vi "Test - Add  Property (Array).vi"() -> ()   [LabVIEW 2020, in "JSON Schema Generator.lvlib"]
uses:
  JSON Schema Generator.lvlib
  <vilib>/addons/_JKI Toolkits/Caraya/classes/Test/Test.lvclass
  <vilib>/addons/_JKI Toolkits/Caraya/classes/Assert/Assert.lvclass
  <vilib>/JDP Science/JSONtext/JSONtext.lvlib
  <vilib>/addons/_JKI Toolkits/Caraya/classes/Assert/Assert Equal Value_Variant.vi
  <vilib>/addons/_JKI Toolkits/Caraya/classes/Assert/Assert Not Error.vi
panel:
  in  "Array 3":enum16{"Test 1", "Test 2", "Test3"}[](array[ring])
  in  "Array 2":string[](array[string])
  in  "Array":T1(array[cluster])
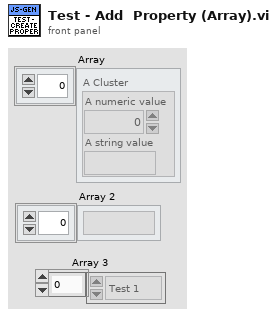
[diagram p1: front panel]
types:
  T1 = cluster{"A numeric value":i32, "A string value":string}[]
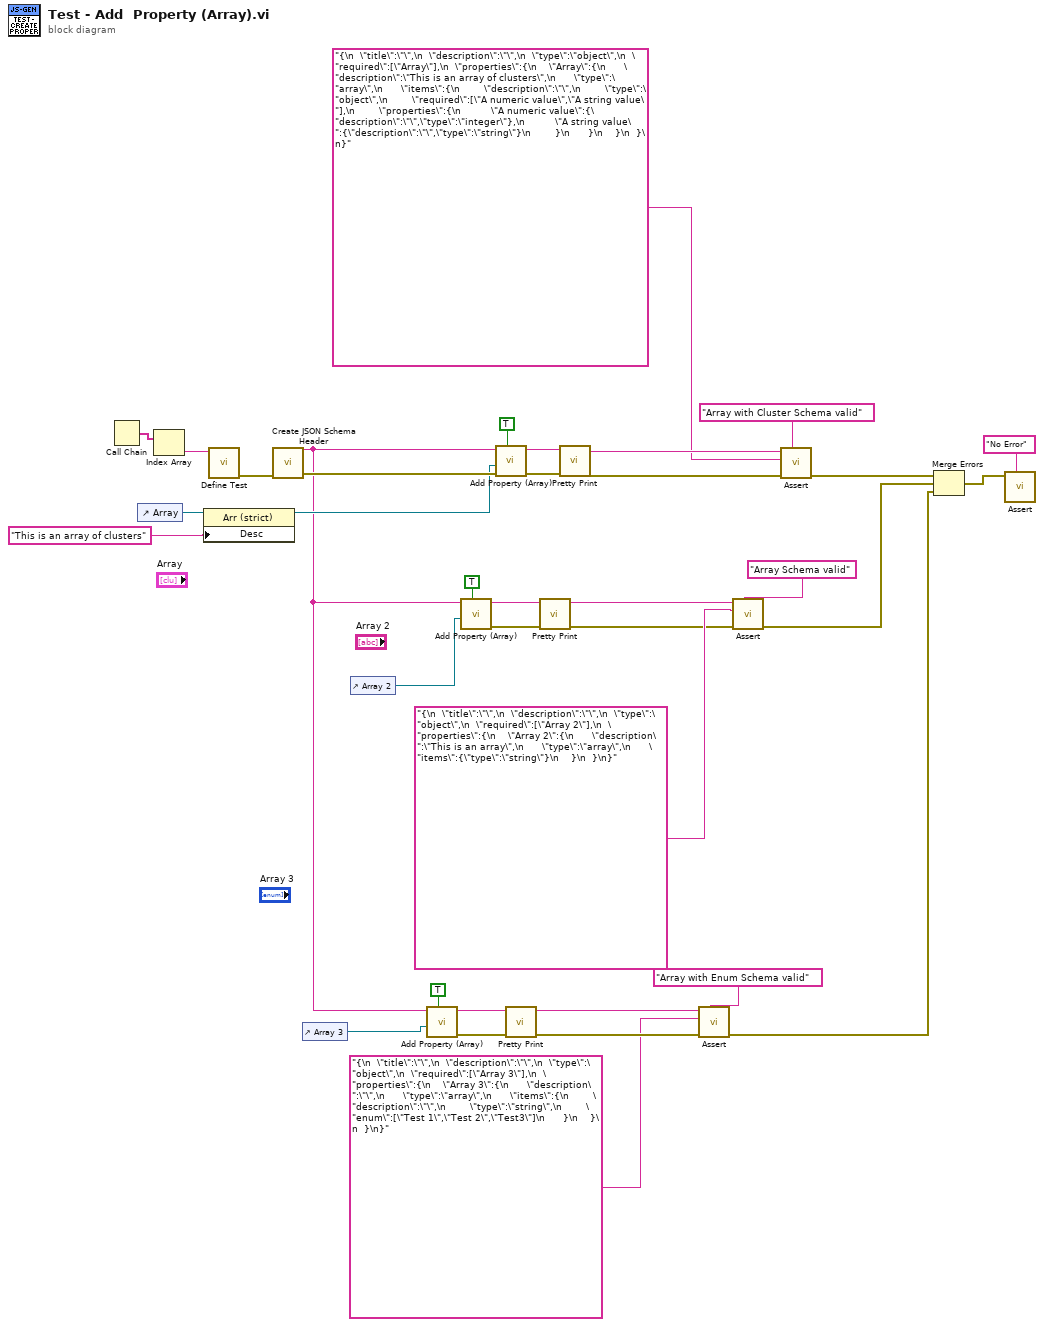
[diagram p0: block diagram]
diagram:
  n1 = Call Chain() -> (call chain=w36:string[])
  n2 = control-ref of="Array"() -> (w17:refnum<vi>)
  n3 = Index Array(array=w36) -> (element=w35:string)  [unwired: 1 in]
  n4 = property on="Property Node" class="Arr (strict)"(reference=w17, "Desc"="This is an array of clusters" ("Description")) -> (reference out=w12:refnum<vi>)  [unwired: 1 in, 1 out]
  n5 = call <vilib>:"Define Test.vi"("Label (VI Title)"=w35) -> ("error out"=w30:errorcluster)  [unwired: 9 in, 1 out]
  n6 = call "Create JSON Schema Header.vi"("error in (no error)"=w30) -> ("error out"=w25:errorcluster, "JSON Schema out"=w1:string)  [unwired: 9 in]
  n7 = control-ref of="Array 3"() -> (w4:refnum<vi>)
  n8 = control-ref of="Array 2"() -> (w16:refnum<vi>)
  n9 = call "Add Property (Array).vi"("Required?"=TRUE, "Array Ref in"=w4, "JSON Schema in"=w1) -> ("error out"=w7:errorcluster, "JSON SChema out"=w9:string)  [unwired: 7 in]
  n10 = call "Add Property (Array).vi"("Required?"=TRUE, "Array Ref in"=w16, "JSON Schema in"=w1) -> ("error out"=w19:errorcluster, "JSON SChema out"=w14:string)  [unwired: 7 in]
  n11 = call "Add Property (Array).vi"("Required?"=TRUE, "error in (no error)"=w25, "Array Ref in"=w12, "JSON Schema in"=w1) -> ("error out"=w27:errorcluster, "JSON SChema out"=w28:string)  [unwired: 6 in]
  n12 = call <vilib>:"Pretty Print.vi"("error in (no error)"=w7, "JSON"=w9) -> ("error out"=w8:errorcluster, "<JSON>"=w10:string)  [unwired: 7 in, 1 out]
  n13 = call <vilib>:"Pretty Print.vi"("error in (no error)"=w19, "JSON"=w14) -> ("error out"=w15:errorcluster, "<JSON>"=w13:string)  [unwired: 7 in, 1 out]
  n14 = call <vilib>:"Pretty Print.vi"("error in (no error)"=w27, "JSON"=w28) -> ("error out"=w26:errorcluster, "<JSON>"=w24:string)  [unwired: 7 in, 1 out]
  n15 = call-poly <vilib>:"Assert.vi"("Label"="Array with Enum Schema valid", "error in (no error)"=w8, "Actual"="{\n  \"title\":\"\",\n  \"description\":\"\",\n  \"type\":\"object\",\n  \"required\":[\"Array 3\"],\n  \"properties\":{\n    \"Array 3\":{\n      \"description\":\"\",\n      \"type\":\"array\",\n      \"items\":{\n        \"description\":\"\",\n        \"type\":\"string\",\n        \"enum\":[\"Test 1\",\"Test 2\",\"Test3\"]\n      }\n    }\n  }\n}", "Expected"=w10) -> ("error out"=w3:errorcluster)  [unwired: 6 in, 1 out]
  n16 = call-poly <vilib>:"Assert.vi"("Label"="Array Schema valid", "error in (no error)"=w15, "Actual"="{\n  \"title\":\"\",\n  \"description\":\"\",\n  \"type\":\"object\",\n  \"required\":[\"Array 2\"],\n  \"properties\":{\n    \"Array 2\":{\n      \"description\":\"This is an array\",\n      \"type\":\"array\",\n      \"items\":{\"type\":\"string\"}\n    }\n  }\n}", "Expected"=w13) -> ("error out"=w18:errorcluster)  [unwired: 6 in, 1 out]
  n17 = call-poly <vilib>:"Assert.vi"("Label"="Array with Cluster Schema valid", "error in (no error)"=w26, "Actual"="{\n  \"title\":\"\",\n  \"description\":\"\",\n  \"type\":\"object\",\n  \"required\":[\"Array\"],\n  \"properties\":{\n    \"Array\":{\n      \"description\":\"This is an array of clusters\",\n      \"type\":\"array\",\n      \"items\":{\n        \"description\":\"\",\n        \"type\":\"object\",\n        \"required\":[\"A numeric value\",\"A string value\"],\n        \"properties\":{\n          \"A numeric value\":{\"description\":\"\",\"type\":\"integer\"},\n          \"A string value\":{\"description\":\"\",\"type\":\"string\"}\n        }\n      }\n    }\n  }\n}", "Expected"=w24) -> ("error out"=w33:errorcluster)  [unwired: 6 in, 1 out]
  n18 = Merge Errors(w33, w18, w3) -> (w31:errorcluster)
  n19 = call-poly <vilib>:"Assert.vi"("Label"="No Error", "Not Error?"=w31) -> ()  [unwired: 8 in, 2 out]
